vi "Get Accounts File Path.vi"(8 "error in":errorcluster) -> (0 "error out":errorcluster, 3 "Accounts File Path":path)   [LabVIEW 2026]
doc: "Returns the absolute path of the ATM accounts file (ATM accounts.txt). The base folder depends on where the VI runs, read from the Application property Kind: in a built application (Run Time System) it is the folder of the exe, from NI's Application Directory.vi (vi.lib\\Utility\\file.llb), where the build specification puts ATM accounts.txt; in the development system (with or without a project) it is two folders above this VI - the folder of the main ATM VI, one above the SubVIs folder that holds this VI. No file dialog is ever shown. error in is passed through unchanged to error out."
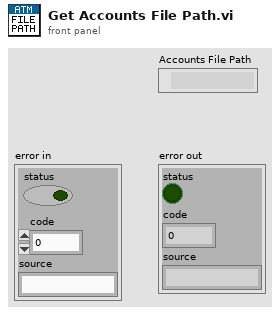
[diagram p1: front panel]
types:
  T1 = enum32{"invalid app kind", "Development System", "Run Time System", "Student Edition", "Embedded LabVIEW", "Evaluation", "Custom"}
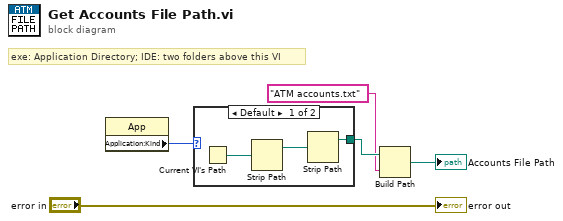
[diagram p0: block diagram]
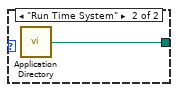
[diagram p2: hidden frame]
diagram:
  # "exe: Application Directory; IDE: two folders above this VI"
  n1 = property class="App"() -> ("Application:Kind"=w4:T1)  [unwired: 2 in, 2 out]
  n2 = case shown="Default" w4 {
    tunnel: [w6 w9] -> w5
    frame Default {
      n3 = Current VI's Path() -> (path=w7:path)
      n4 = Strip Path(path=w7) -> (stripped path=w8:path)  [unwired: 1 out]
      n5 = Strip Path(path=w8) -> (stripped path=w6:path)  [unwired: 1 out]
    }
    frame "Run Time System" {
      n6 = call <vilib>:"Application Directory.vi"() -> ("Application Directory"=w9:path)
    }
  }
  n7 = Build Path(base path=w5, name or relative path="ATM accounts.txt" ("Accounts File Name")) -> (appended path=→"Accounts File Path":path)
  "error out" <- "error in"
